vi "Qualified Name - When Not Constructed - Is Empty.vi"() -> ()   [LabVIEW 2017, in "Test Case.Tests.lvlib"]
uses:
  Test Case.Tests.lvlib
  Test Case/Test Case.lvclass
  Test Case/Test Case.lvclass/Test Case.ctl
  Test Case/Get Qualified Name.vi
  <vilib>/PNR/Transparent Assertions/Transparent Assertions/Transparent Assertions.lvlib
panel:
  out "error out":errorcluster
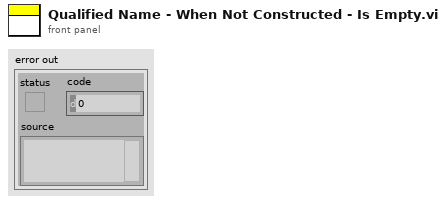
[diagram p1: front panel]
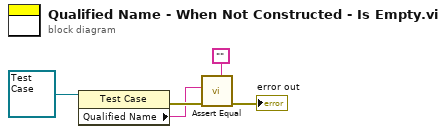
[diagram p0: block diagram]
diagram:
  n1 = property class="Test Case"(reference=refnum<class "Test Case.lvclass"> refnum ("Test Case")) -> (error out=w4:errorcluster, "Qualified Name"=w3:string)  [unwired: 1 in, 1 out]
  n2 = call <vilib>:"Assert Equal.vi"("Expected"="", "error in (no error)"=w4, "Actual"=w3) -> ("error out"=→"error out":errorcluster)  [unwired: 8 in]
